vi "array dinension - template.vi"() -> ()   [LabVIEW 2012]
panel:
  out "Array Size":i32
  in  "Index":i32
  in  "Array":dbl[][](array[numeric])
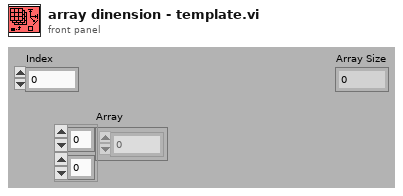
[diagram p1: front panel]
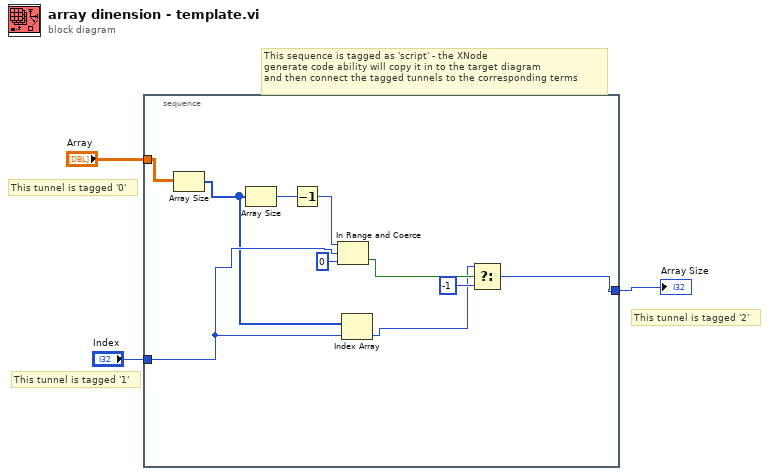
[diagram p0: block diagram]
diagram:
  # "This tunnel is tagged '2'"
  # "This tunnel is tagged '1'"
  # "This tunnel is tagged '0'"
  # "This sequence is tagged as 'script' - the XNode \ngenerate code ability will copy it in to the target diagram\nand then connect the tagged tunnels to the corresponding terms"
  n1 = stacked-sequence {
    tunnel: "Array" -> [w5]
    tunnel: "Index" -> [w12]
    tunnel: [w9] -> w1
    frame #0 {
      n2 = Array Size(array=w5) -> (size(s)=w4:i32[])
      n3 = Array Size(array=w4) -> (size(s)=w7:i32)
      n4 = Decrement(x=w7) -> (x-1=w6:i32)
      n5 = In Range and Coerce(upper limit=w6, x=w12, lower limit=0) -> (In Range?=w11:bool)  [unwired: 1 out]
      n6 = Index Array(array=w4, index=w12) -> (element=w8:i32)
      n7 = Select(t=w8, s=w11, f=-1) -> (s? t:f=w9:i32)
    }
  }
  "Array Size" <- w1
